vi "PackageNode_Create.vi"(0 "reference":refnum<class "PackageNode.lvclass">, 5 "error in (no error)":errorcluster) -> (14 "reference out":refnum<class "PackageNode.lvclass">, 19 "error out":errorcluster)   [LabVIEW 2020, in "PackageNode.lvclass"]
doc: "Creates and initializes a new PackageNode object.\n\nThis object should be destroyed using a PackageNode destructor VI or a virtual base class destructor VI.\n\n[GOOP 2.1]"
uses:
  <resource>/Framework/Providers/Open_GDS/UML/PackageNode_class/PackageNode.lvclass
  C:/Program Files (x86)/National Instruments/LabVIEW 2020/resource/Framework/Providers/Open_GDS/UML/RectangularNode_class/RectangularNode.lvclass
  <resource>/Framework/Providers/Open_GDS/UML/RectangularNode_class/RectangularNode.lvclass
  <resource>/Framework/Providers/Open_GDS/UML/MultiLineString_class/MultiLineString.lvclass
panel:
  # "The input reference should only\nbe wired when this method is called\nby a sub class constructor."
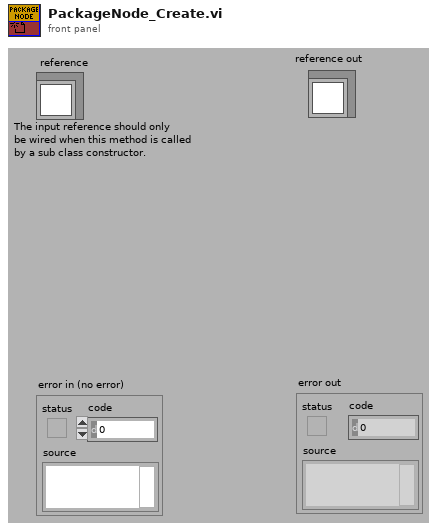
[diagram p1: front panel]
types:
  T1 = typedef "PackageNode.lvclass/ObjectAttributes.ctl" = cluster{"name":string, "contents":refnum<class "MultiLineString.lvclass">, "DEFAULT_TOP_WIDTH":i32, "DEFAULT_TOP_HEIGHT":i32, "DEFAULT_WIDTH":i32, "DEFAULT_HEIGHT":i32, "NAME_GAP":i32, "XGAP":i32, "YGAP":i32, "Collapsed":bool, "Note color":u32, "Justification":u16}
  T2 = typedef "RectangularNode.lvclass/ObjectAttributes.ctl" = cluster{"bounds":T3}
  T3 = typedef "Rectangle Rectangle2D.ctl" = cluster{"x":dbl, "y":dbl, "width":dbl, "height":dbl}
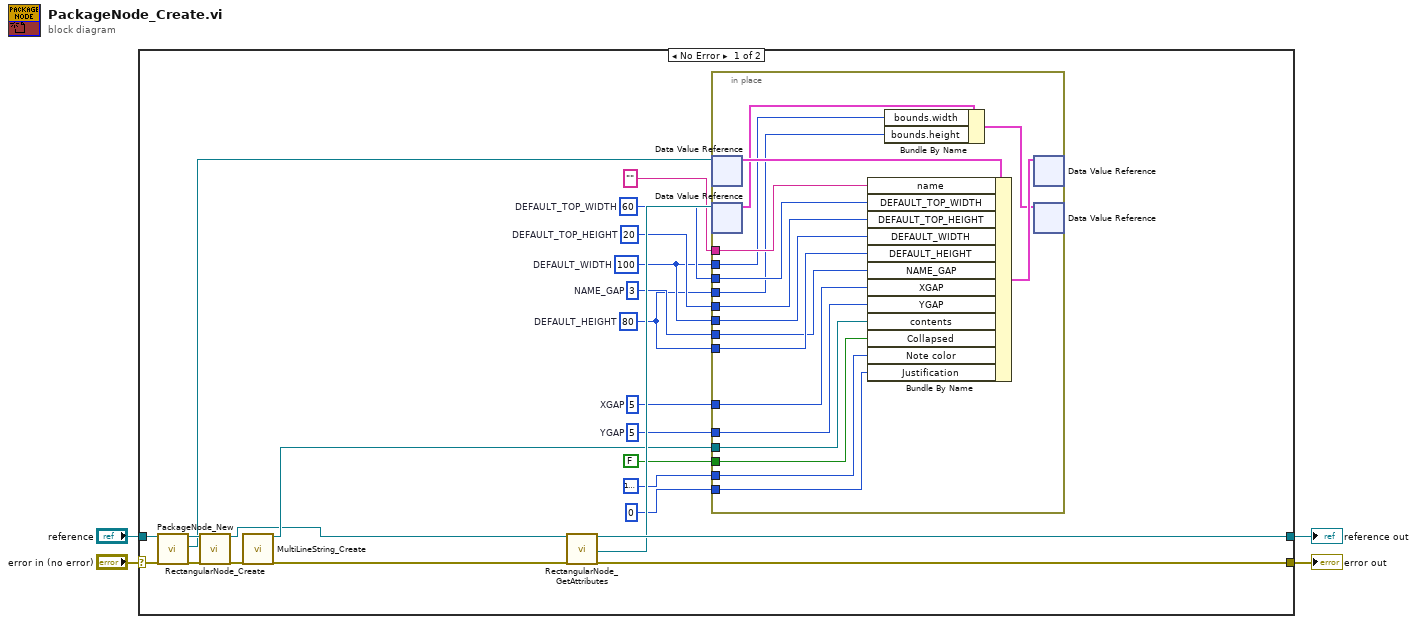
[diagram p0: block diagram]
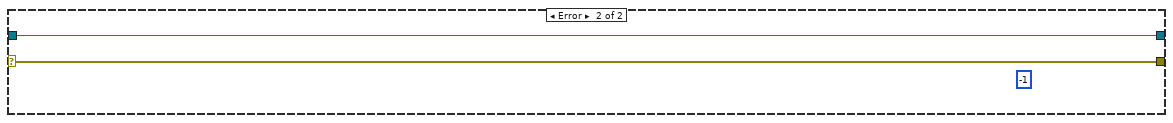
[diagram p2: hidden frame]
diagram:
  n1 = case shown="No Error" "error in (no error)" {
    selector: "error in (no error)" -> [w27 w47]
    tunnel: [w23 w46] -> w4
    tunnel: [w22 w47] -> w3
    tunnel: "reference" -> [w26 w46]
    frame No Error {
      w14 = 5  # YGAP
      w15 = 5  # XGAP
      w16 = 3  # NAME_GAP
      w8 = 80  # DEFAULT_HEIGHT
      w9 = 100  # DEFAULT_WIDTH
      w17 = 20  # DEFAULT_TOP_HEIGHT
      w18 = 60  # DEFAULT_TOP_WIDTH
      n2 = call <resource>:"PackageNode_New.vi"("reference in"=w26, "error in (no error)"=w27) -> ("reference out"=w24:refnum<class "PackageNode.lvclass">, "DVRRefOut"=w7:refnum<data-value>, "error out"=w25:errorcluster)  [unwired: 2 in, 13 out]
      n3 = call <resource>:"RectangularNode_Create.vi"("reference"=w24, "error in (no error)"=w25) -> ("reference out"=w6:refnum<class "PackageNode.lvclass">, "error out"=w21:errorcluster)  [unwired: 1 in, 15 out]
      n4 = call <resource>:"MultiLineString_Create.vi"("error in (no error)"=w21) -> ("reference out"=w13:refnum<class "MultiLineString.lvclass">, "error out"=w5:errorcluster)  [unwired: 2 in, 15 out]
      n5 = call <resource>:"RectangularNode_GetAttributes.vi"("reference in"=w6, "error in (no error)"=w5) -> ("reference out"=w23:refnum<class "PackageNode.lvclass">, "DataRef"=w20:refnum<data-value>, "error out"=w22:errorcluster)  [unwired: 14 in, 1 out]
      n6 = in-place {
        in-place-border: "" ("name") -> [w44]
        in-place-border: w18 -> [w43]
        in-place-border: w17 -> [w42]
        in-place-border: w9 -> [w41]
        in-place-border: w8 -> [w40]
        in-place-border: w16 -> [w39]
        in-place-border: w15 -> [w38]
        in-place-border: w14 -> [w37]
        in-place-border: w13 -> [w36]
        in-place-border: FALSE ("Collapsed") -> [w35]
        in-place-border: u32 16777216 -> [w34]
        in-place-border: u16 0 ("Justification") -> [w33]
        in-place-border: w9 -> [w30]
        in-place-border: w8 -> [w29]
        n7 = in-place-dvr #1(w7) -> (w45:T1)  [unwired: 1 out]
        n8 = in-place-dvr #2(w20) -> (w31:T2)  [unwired: 1 out]
        n9 = Bundle By Name(cluster=w45, "name"=w44, "DEFAULT_TOP_WIDTH"=w43, "DEFAULT_TOP_HEIGHT"=w42, "DEFAULT_WIDTH"=w41, "DEFAULT_HEIGHT"=w40, "NAME_GAP"=w39, "XGAP"=w38, "YGAP"=w37, "contents"=w36, "Collapsed"=w35, "Note color"=w34, "Justification"=w33) -> (w32:T1)
        n10 = Bundle By Name(cluster=w31, "bounds.width"=w30, "bounds.height"=w29) -> (w28:T2)
        n11 = in-place-dvr #1(w32) -> ()  [unwired: 2 out]
        n12 = in-place-dvr #2(w28) -> ()  [unwired: 2 out]
      }
    }
    frame Error {
      (unwired) -1 ("Nr of open handles")
    }
  }
  "error out" <- w3
  "reference out" <- w4
